vi "Initialize.vi"(7 "Time Entry Store in":refnum<class "Time Entry Store.lvclass">, 8 "error in (no error)":errorcluster, 11 "Data Folder":path) -> (0 "error out":errorcluster, 5 "Time Entry Store out":refnum<class "Time Entry Store.lvclass">)   [LabVIEW 2024, in "Time Entry Store.lvclass"]
doc: "Prepares the store to use the given data folder. The parent class has no storage: it returns empty results and does nothing. Time Entry Store-INI overrides it.\n\nGenerated by: Claude"
uses:
  Time Entry Store.lvclass
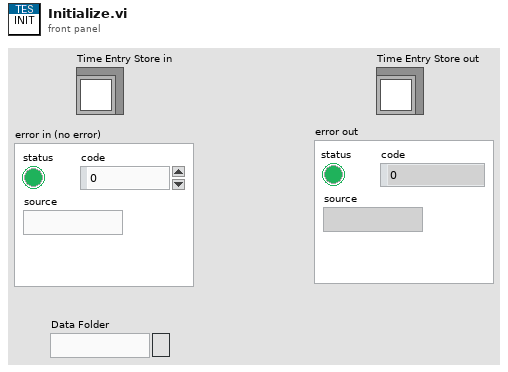
[diagram p1: front panel]
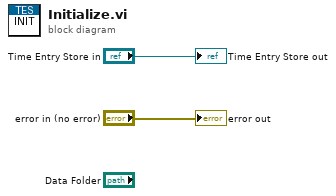
[diagram p0: block diagram]
diagram:
  "Time Entry Store out" <- "Time Entry Store in"
  "error out" <- "error in (no error)"
